vi "子VI-Close.vi"(0 "会话":u32=4294967295) -> (1 "返回值":u32, 2 "描述":string)   [LabVIEW 2011]
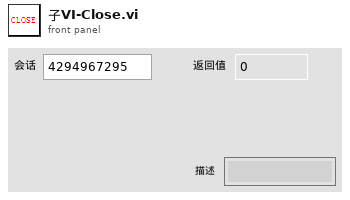
[diagram p1: front panel]
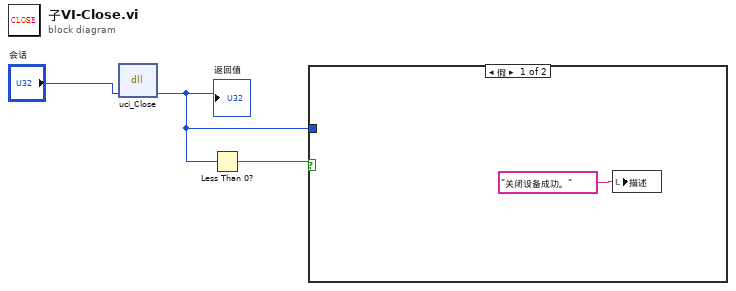
[diagram p0: block diagram]
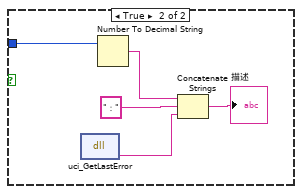
[diagram p2: hidden frame]
diagram:
  n1 = dll-call lib="PTH1Eabs E调试程序\nLabView程序UCI示例程序ASCIIuci.dll" fn="uci_Close"("session"="会话") -> ("session"=w1:u32)  [unwired: 4 in, 2 out]
  "返回值" <- w1
  n2 = Less Than 0?(x=w1) -> (x < 0?=w2:bool)
  n3 = case shown="假" w2 {
    tunnel: w1 -> [_ w5]
    frame False {
      n4 = local write "描述"("关闭设备成功。") -> ()
    }
    frame True {
      n5 = dll-call lib="PTH1Eabs E调试程序\nLabView程序UCI示例程序ASCIIuci.dll" fn="uci_GetLastError"() -> ("返回类型"=w7:string)  [unwired: 3 in, 2 out]
      n6 = Number To Decimal String(number=w5) -> (decimal integer string=w9:string)  [unwired: 1 in]
      n7 = Concatenate Strings(w9, "：", w7) -> (→"描述":string)
    }
  }
